vi "Lab3_KS.vi"() -> ()   [LabVIEW 2025]
uses:
  Runners_Data.ctl
  HR_Data_Structure.ctl
  Raw_Data.ctl
panel:
  out "error out":errorcluster
  in  "error in":errorcluster
  in  "File Path":path
  in  "HR":T1={"Runners_Data"={"Name"="", "Age"=0}, "HR Max"=0, "Cluster"={"Time"=[], "Bpm"=[]}, "% HR MAX"=[], "Total Time In Zone"=[], "Zones info"=[["Z1", "Endurance"], ["Z2", "Moderate"], ["Z3", "Tempo"], ["Z4", "Threshold"], ["Z5", "Anaerobic"]], "Heart Rate Zone No"=[]}
  in  "Cluster":T2
  out "HEART RATE ZONES":string[][](array[string])
  out "XY Graph":T4(graph)
  out "BPM":cluster{"Time":timestamp[], "Bpm":i32[]}(graph)
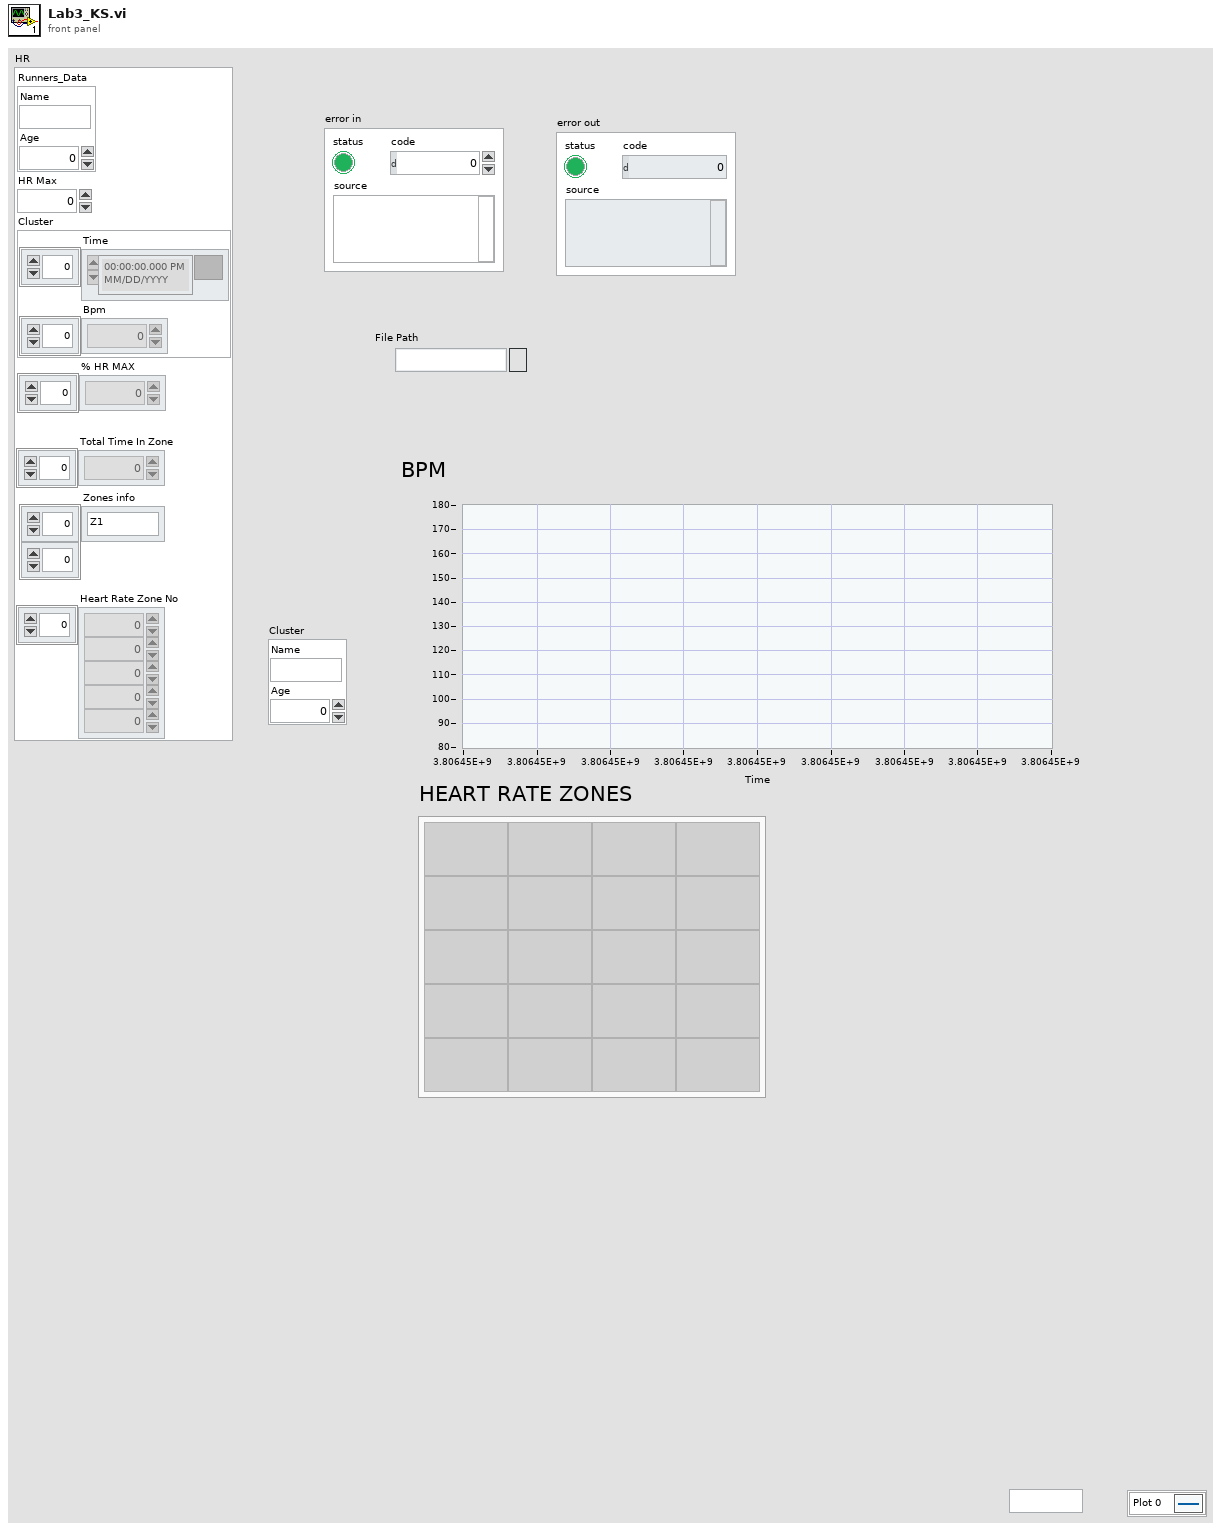
[diagram p1: front panel]
types:
  T1 = typedef "HR_Data_Structure.ctl" = cluster{"Runners_Data":T2, "HR Max":i32, "Cluster":T3, "% HR MAX":dbl[], "Total Time In Zone":dbl[], "Zones info":string[][], "Heart Rate Zone No":dbl[]}
  T2 = typedef "Runners_Data.ctl" = cluster{"Name":string, "Age":i32}
  T3 = typedef "Raw_Data.ctl" = cluster{"Time":timestamp[], "Bpm":i32[]}
  T4 = cluster{"Total Time In Zone":dbl[], "Heart Rate Zone No":dbl[]}
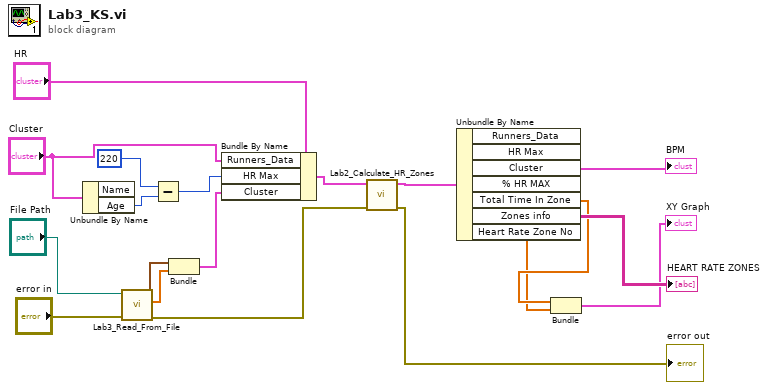
[diagram p0: block diagram]
diagram:
  n1 = Unbundle By Name("Cluster") -> ("Age"=w19:i32)  [unwired: 1 out]
  n2 = call "Lab3_Read_From_File.vi"("error in"="error in", "File Path"="File Path") -> ("error out"=w15:errorcluster, "Array"=w12:dbl[], "Array 2"=w11:timestamp[])  [unwired: 7 in]
  n3 = Subtract(x=220, y=w19) -> (x-y=w9:i32)
  n4 = Bundle("Array 2"=w11, "Array"=w12) -> (w10:cluster{"Array 2":timestamp[], "Array":dbl[]})  [unwired: 1 in]
  n5 = Bundle By Name(cluster="HR", "Runners_Data"="Cluster", "HR Max"=w9, "Cluster"=w10) -> (w7:T1)
  n6 = call "Lab2_Calculate_HR_Zones.vi"("error in (no error)"=w15, "HR_IN"=w7) -> ("error out"=→"error out":errorcluster, "HR_OUT"=w6:T1)  [unwired: 8 in]
  n7 = Unbundle By Name(w6) -> ("Cluster"=→"BPM":T3, "Total Time In Zone"=w3:dbl[], "Zones info"=→"HEART RATE ZONES":string[][], "Heart Rate Zone No"=w2:dbl[])  [unwired: 3 out]
  n8 = Bundle "Bundle"("Total Time In Zone"=w3, "Heart Rate Zone No"=w2) -> (→"XY Graph":T4)  [unwired: 1 in]
